vi "CIVI Initialize Close Example.vi"() -> ()   [LabVIEW 2026]
panel:
  out "SCPI Error Code":i32
  out "Frequency Response":string
  out "IDN Response":string
  out "error out":errorcluster
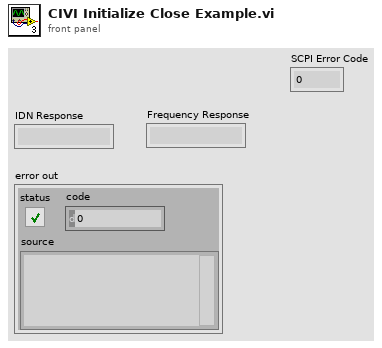
[diagram p1: front panel]
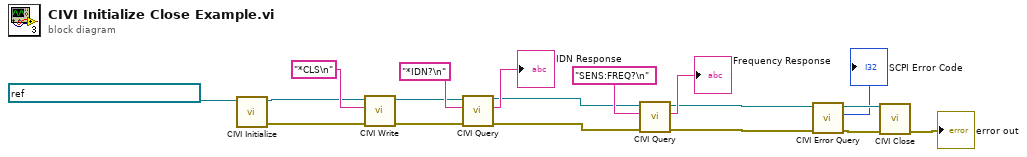
[diagram p0: block diagram]
diagram:
  n1 = call "CIVI Initialize.vi"("VISA Resource Name"=refnum<visa-resource-name> "TCPIP0::127.0.0.1::5025::SOCKET") -> ("error out"=w10:errorcluster, "VISA Session out"=w6:refnum<visa-resource-name>)  [unwired: 9 in]
  n2 = call "CIVI Write.vi"("error in"=w10, "write buffer"="*CLS\n", "VISA Session in"=w6) -> ("error out"=w8:errorcluster, "VISA Session out"=w9:refnum<visa-resource-name>)  [unwired: 7 in]
  n3 = call "CIVI Query.vi"("error in"=w8, "write buffer"="*IDN?\n", "VISA Session in"=w9) -> ("error out"=w11:errorcluster, "read buffer"=→"IDN Response":string, "VISA Session out"=w12:refnum<visa-resource-name>)  [unwired: 6 in]
  n4 = call "CIVI Query.vi"("error in"=w11, "write buffer"="SENS:FREQ?\n", "VISA Session in"=w12) -> ("error out"=w2:errorcluster, "read buffer"=→"Frequency Response":string, "VISA Session out"=w4:refnum<visa-resource-name>)  [unwired: 6 in]
  n5 = call "CIVI Error Query.vi"("error in"=w2, "VISA Session in"=w4) -> ("error out"=w3:errorcluster, "SCPI Error Code"=→"SCPI Error Code":i32, "VISA Session out"=w5:refnum<visa-resource-name>)  [unwired: 7 in]
  n6 = call "CIVI Close.vi"("error in"=w3, "VISA Session in"=w5) -> ("error out"=→"error out":errorcluster)  [unwired: 9 in]
